vi "VM - Not a VC Handle.vi"(0 "VC Handle":T1=-1) -> (2 "Not a VC Handle":bool)   [LabVIEW 2021]
doc: "This VI returns TRUE if <b>VC Handle</b> is not a valid variable context handle. Refer to the VI help for more details.\n\n::: CalcExpress Toolkit :::\nCopyright (c) 2000-2026 Konstantin Shifershteyn. All rights reserved."
uses:
  cetypes.llb/VarMan Variable Context Handle.ctl
  cersrc/celveng32.dll
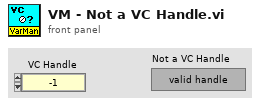
[diagram p1: front panel]
types:
  T1 = typedef "VarMan Variable Context Handle.ctl" = i32
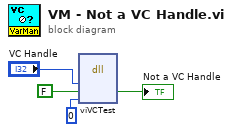
[diagram p0: block diagram]
diagram:
  n1 = dll-call lib="C:/LV Projects/CalcExpress 40 LV2021/vi.lib/addons/CalcExpress/cersrc/celveng*.dll" fn="viVCTest"("vch"="VC Handle", "errf"=FALSE, "errc"=u16 0) -> ("errf"=→"Not a VC Handle":bool)  [unwired: 6 in, 2 out]
